vi "Highlight.vi"() -> ()   [LabVIEW 2017]
uses:
  <vilib>/Utility/traverseref.llb/TRef TravTarget.ctl
  user.lib/_NEVSTOP/Communicable State Machine(CSM)/_Polymophic/Add State(s) to Queue By BOOL(Element).vi
  user.lib/_NEVSTOP/Communicable State Machine(CSM)/Communicable State Machine.lvlib
  <vilib>/Utility/traverseref.llb/VI Scripting - Traverse.lvlib
panel:
  in  "Highlight All Scripts":bool
  in  "Highlight Scripts":bool
  out "String":string
  in  "Listbox":i32(listbox)
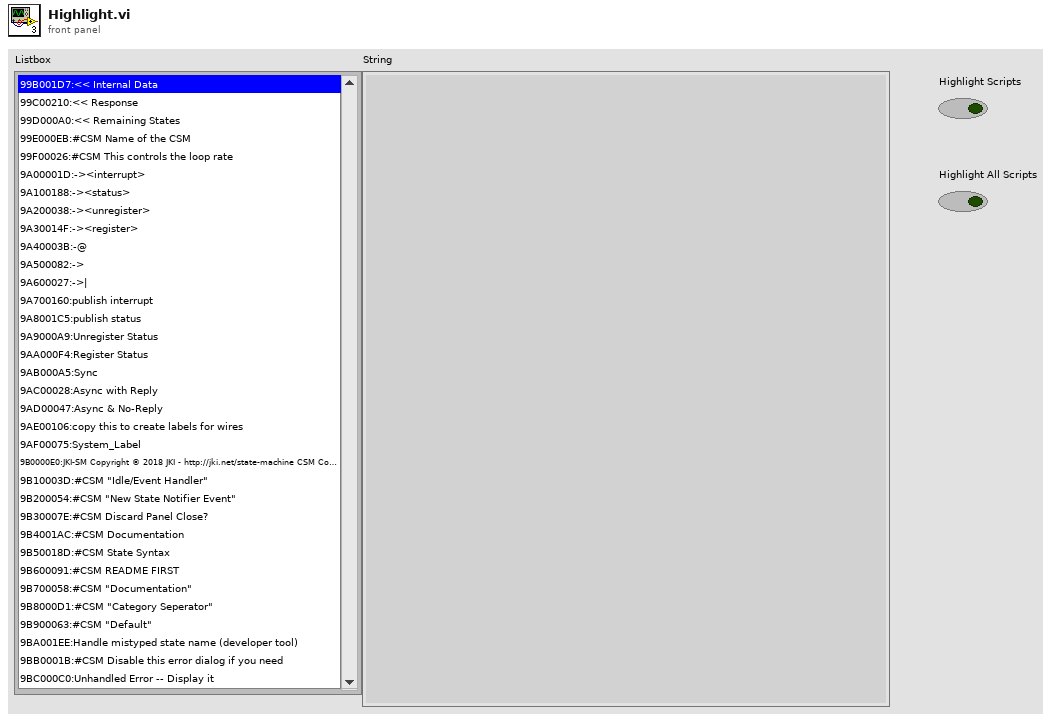
[diagram p1: front panel]
types:
  T1 = enum32{"Invalid", "Standard", "Closed", "Hidden", "Minimized", "Maximized"}
  T2 = enum32{"invalid app kind", "Development System", "Run Time System", "Student Edition", "Embedded LabVIEW", "Evaluation", "Custom"}
  T3 = typedef "TRef TravTarget.ctl" = enum16{"FP", "BD", "Other"}
  T4 = cluster{"Core":cluster{"Current VI Reference":refnum<vi>, "Close Panel on Exit?":bool}, "VI":path, "VIRef":refnum<vi>}
  T5 = cluster{"Current VI Reference":refnum<vi>, "Close Panel on Exit?":bool}
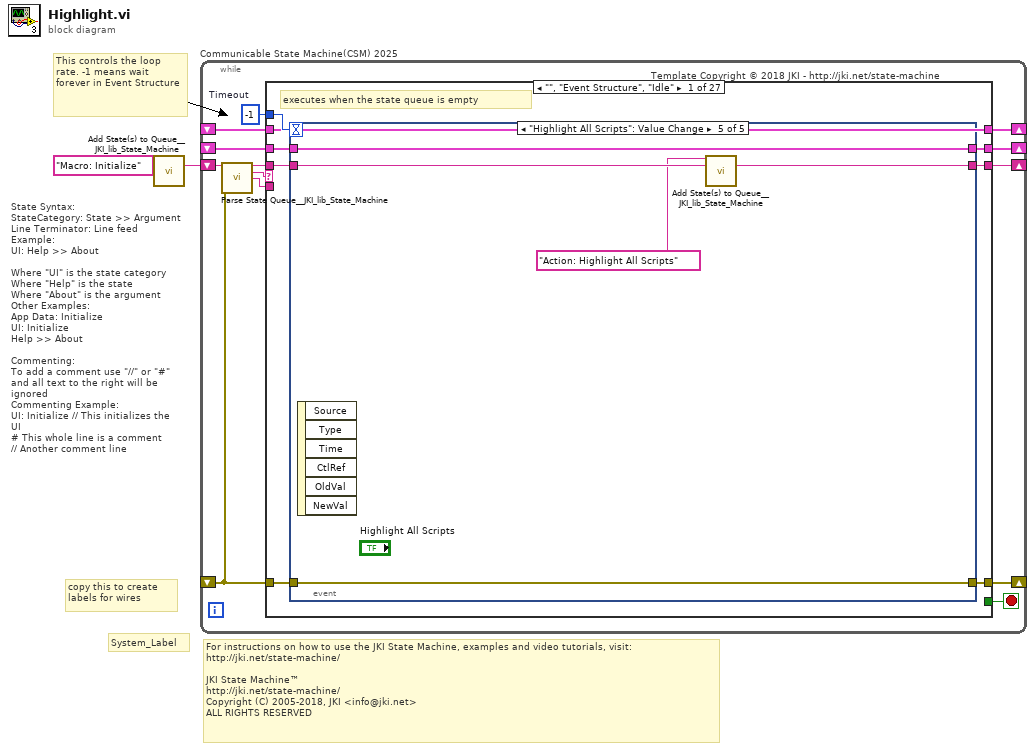
[diagram p0: block diagram]
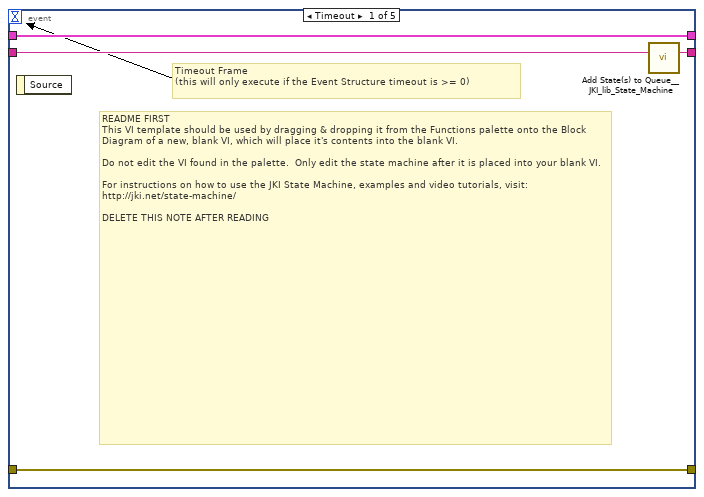
[diagram p2: hidden frame]
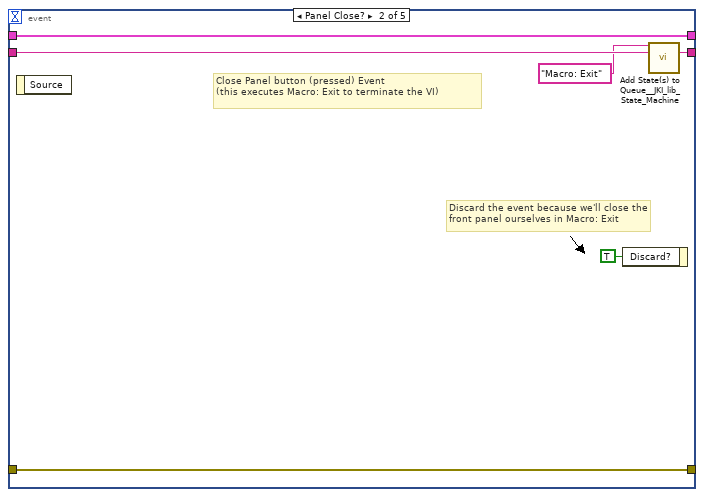
[diagram p3: hidden frame]
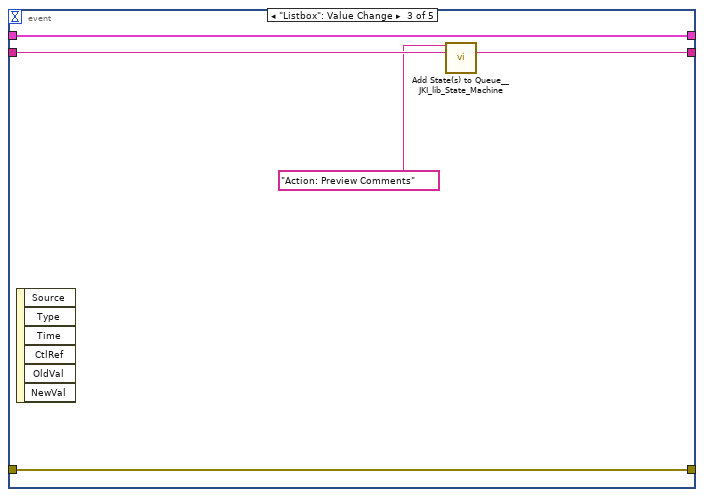
[diagram p4: hidden frame]
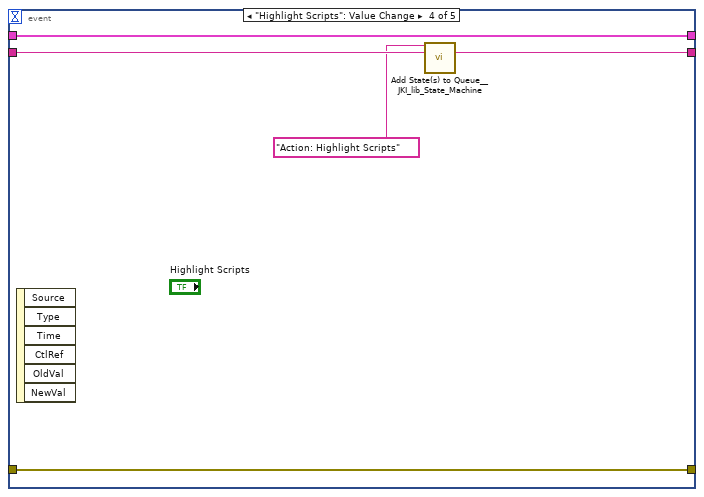
[diagram p5: hidden frame]
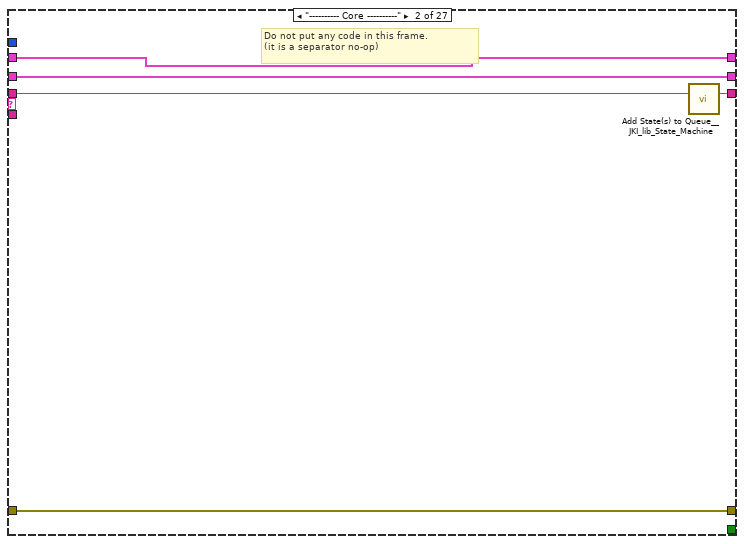
[diagram p6: hidden frame]
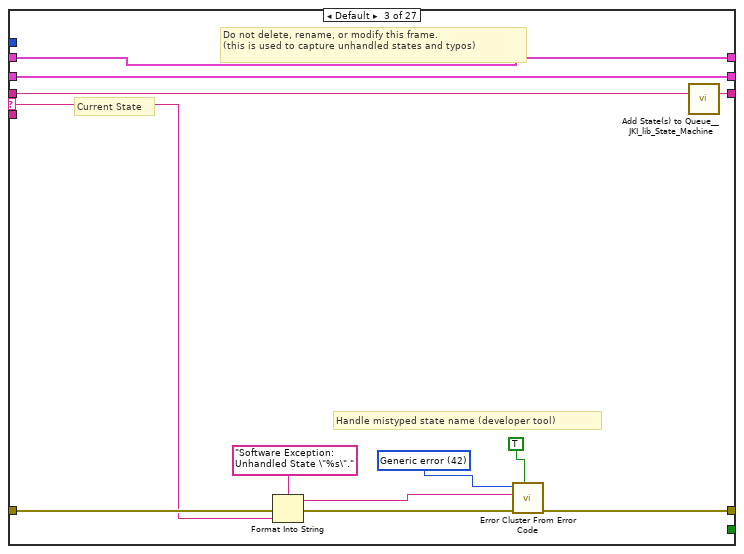
[diagram p7: hidden frame]
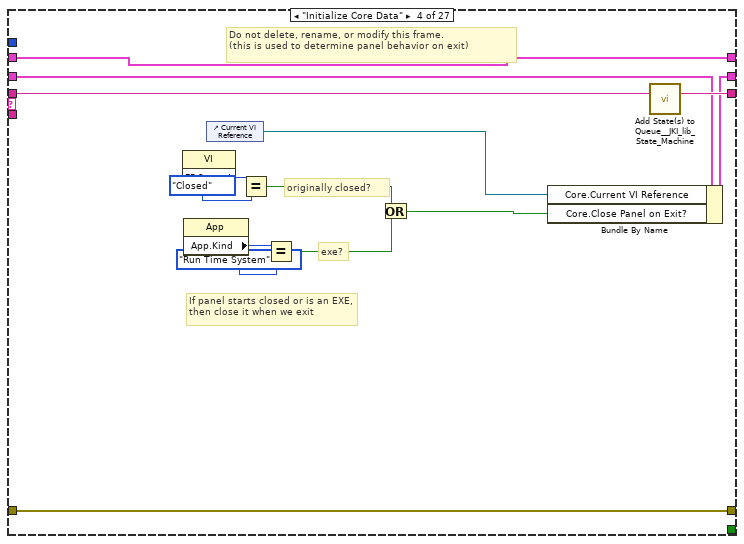
[diagram p8: hidden frame]
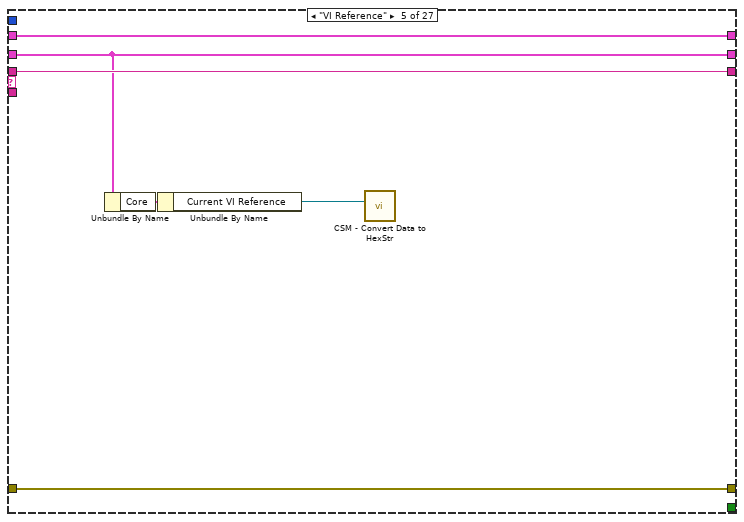
[diagram p9: hidden frame]
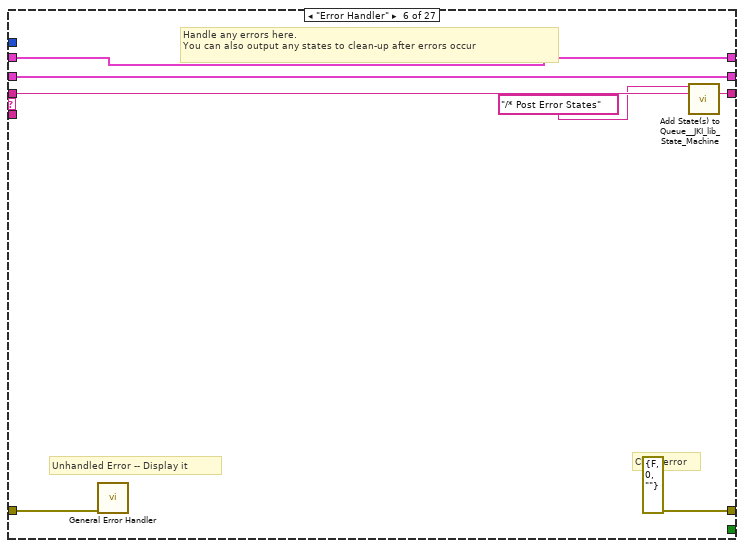
[diagram p10: hidden frame]
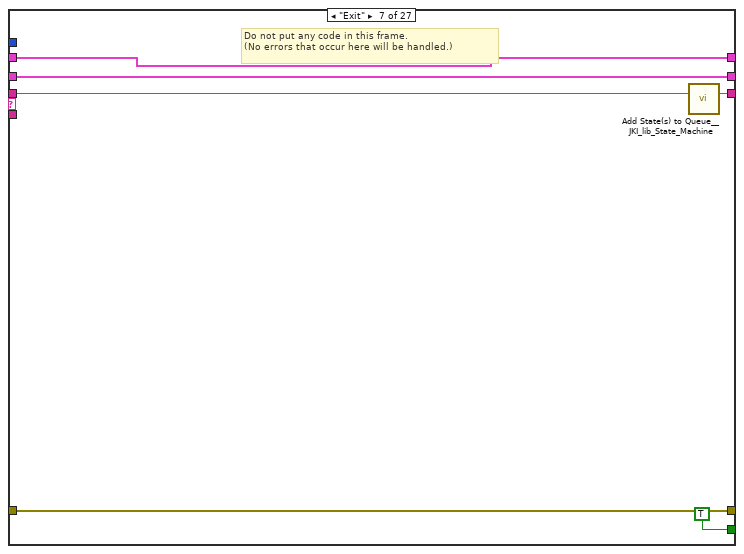
[diagram p11: hidden frame]
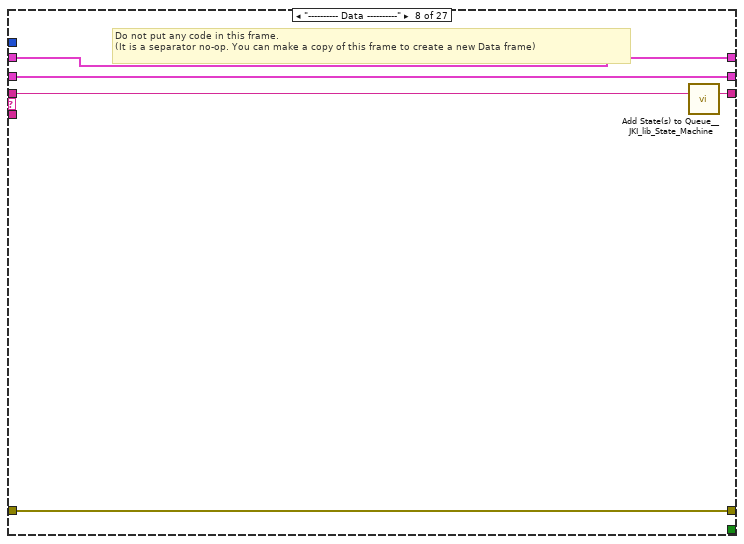
[diagram p12: hidden frame]
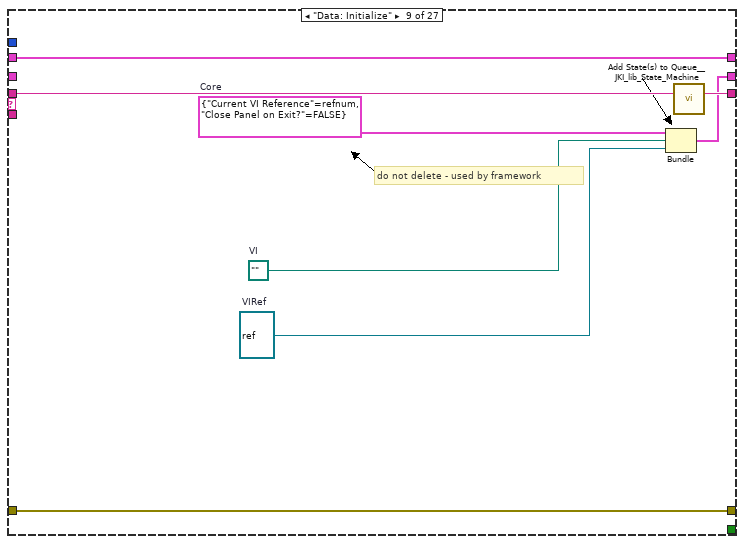
[diagram p13: hidden frame]
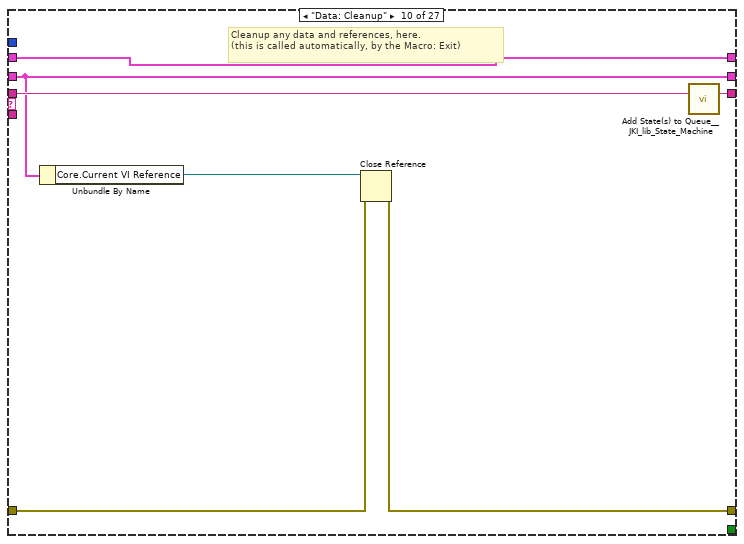
[diagram p14: hidden frame]
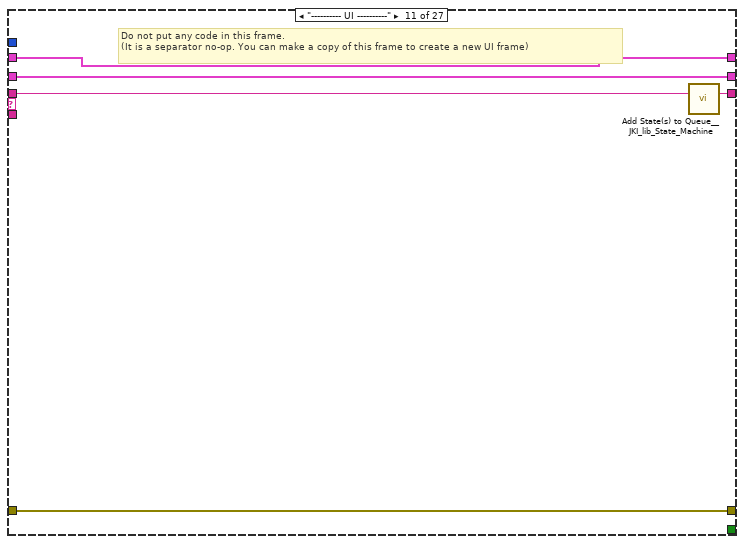
[diagram p15: hidden frame]
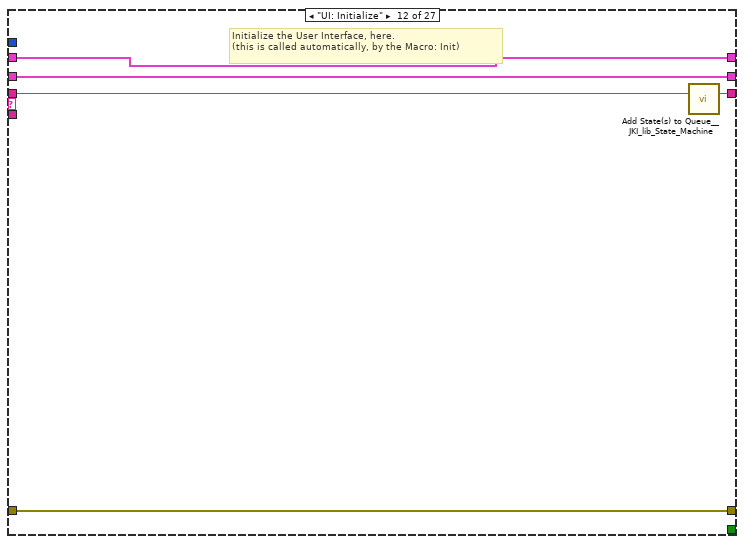
[diagram p16: hidden frame]
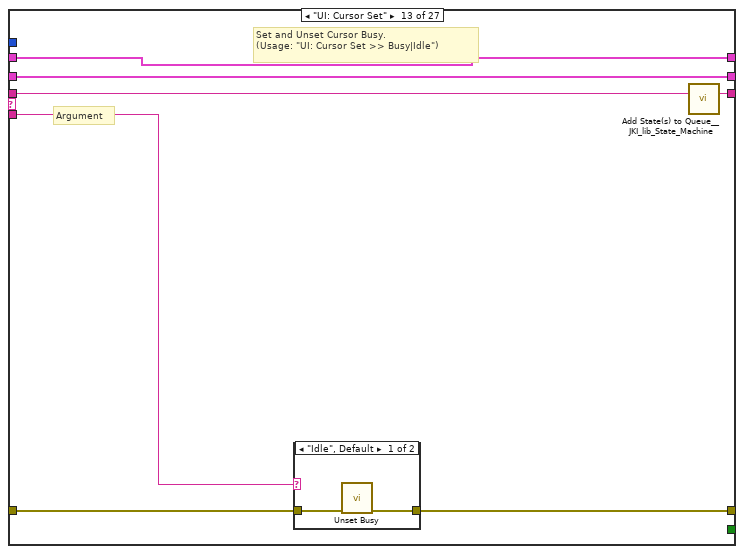
[diagram p17: hidden frame]
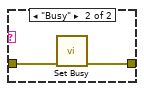
[diagram p18: hidden frame]
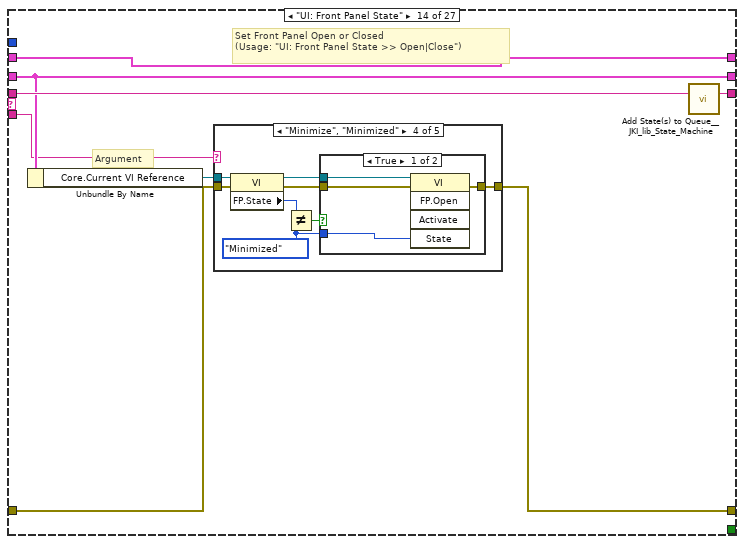
[diagram p19: hidden frame]
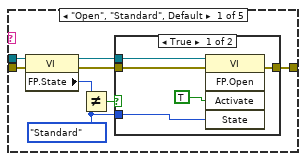
[diagram p20: hidden frame]
diagram:
  # "For instructions on how to use the JKI State Machine, examples and video tutorials, visit:\nhttp://jki.net/state-machine/\n\nJKI State Machine™\nhttp://jki.net/state-machine/\nCopyright (C) 2005-2018, JKI <info@jki.net>\nALL RIGHTS RESERVED"
  # "State Syntax:\nStateCategory: State >> Argument\nLine Terminator: Line feed\nExample:\nUI: Help >> About\n\nWhere \"UI\" is the state category\nWhere \"Help\" is the state\nWhere \"About\" is the argument\nOther Examples:\nApp Data: Initialize\nUI: Initialize\nHelp >> About\n\nCommenting:\nTo add a comment use \"//\" or \"#\" and all text to the right will be ignored\nCommenting Example:\nUI: Initialize // This initializes the UI\n# This whole line is a comment\n// Another comment line"
  # "copy this to create labels for wires"
  # "This controls the loop rate. -1 means wait forever in Event Structure"
  # "System_Label"
  n1 = call <vilib>:"Add State(s) to Queue__JKI_lib_State_Machine.vi"("State(s) in (\"\")"="Macro: Initialize") -> ("States Out"=w1:string)  [unwired: 14 in]
  n2 = while "Communicable State Machine(CSM) 2025" {
    shift-right: [w8] -> _
    shift-left: _ -> [w7]
    shift-right: [w11] -> _
    shift-left: _ -> [w5]
    shift-right: [w10] -> _
    shift-left: w1 -> [w12]
    shift-right: [w4] -> _
    shift-left: _ -> [w3]
    stop <- w9 stop-if-true
    w6 = -1  # Timeout
    # "Template Copyright © 2018 JKI - http://jki.net/state-machine"
    n3 = call <vilib>:"Parse State Queue__JKI_lib_State_Machine.vi"("State Queue"=w12, "Error In (no error)"=w5) -> ("Remaining States"=w14:string, "Current State"=w15:string, "Arguments"=w13:string)  [unwired: 11 in]
    n4 = case shown="\"\", \"Event Structure\", \"Idle\"" w15 {
      selector: w15 -> [_ _ w55 _ _ _ _ _ _ _ _ _ _ _ _ _ _ _ _ _ _ _ _ _ _ _ _]
      tunnel: w14 -> [w23 w53 w59 w79 w84 w92 w98 w103 w111 w118 w123 w128 w135 w147 w217 w223 w226 w240 w245 w257 w265 w276 w297 w311 w327 w343 w347]
      tunnel: w13 -> [_ _ _ _ _ _ _ _ _ _ _ _ w130 w141 _ _ _ _ _ _ _ _ _ _ _ _ _]
      tunnel: w7 -> [w21 w50 w57 w72 w83 w89 w96 w100 _ w113 w120 w126 w133 w143 w214 w220 w228 w237 w242 w254 w263 w275 w296 w310 w326 w342 w346]
      tunnel: [w20 w51 w61 w76 w85 errorcluster {"status"=FALSE, "code"=0, "source"=""} ("error out") w95 w101 w108 w114 w121 w125 w131 w144 w215 w221 w229 w238 w243 w255 w266 w277 w298 w312 w328 w333 w345] -> w11
      tunnel: w5 -> [w19 w51 w60 w76 w85 w88 w95 w101 w108 w115 w121 w125 w132 w145 w215 w221 w229 w238 w243 w255 w266 w277 w298 w312 w328 w333 w345]
      tunnel: [w22 w52 w58 w78 w84 w91 w97 w102 w110 w117 w122 w127 w134 w146 w216 w222 w227 w239 w244 w256 w265 w276 w297 w311 w327 w343 w347] -> w10
      tunnel: [_ _ _ _ _ _ TRUE _ _ _ _ _ _ _ _ _ _ _ _ _ _ _ _ _ _ _ _] -> w9
      tunnel: [w18 w50 w57 w77 w83 w89 w96 w100 w109 w113 w120 w126 w133 w143 w214 w220 w228 w237 w242 w248 w261 w275 w296 w310 w326 w342 w346] -> w8
      tunnel: w6 -> [w17 _ _ _ _ _ _ _ _ _ _ _ _ _ _ _ _ _ _ _ _ _ _ _ _ _ _]
      tunnel: [w16 w49 w54 w66 w82 w86 w93 w99 w104 w112 w119 w124 w129 w140 w213 w218 w224 w230 w241 w246 cluster{refnum<vi>, "Text.Text":string}[] [] w267 w287 w308 w323 w339 w344] -> w4
      tunnel: w3 -> [w16 w49 w54 w66 w82 w86 w93 w99 w104 w112 w119 w124 w129 w140 w213 w218 w224 w230 w241 w246 _ w268 w288 w308 w323 w339 w344]
      frame "", "Event Structure", "Idle" {
        # "executes when the state queue is empty"
        n5 = event shown="[4] \"Highlight All Scripts\": Value Change" {
          selector: _ -> [_ _ _ _ _]
          dyn-events: _ -> [_ _ _ _ _]
          timeout: w17 -> [_ _ _ _ _]
          tunnel: w23 -> [w27 w33 w35 w40 w45]
          tunnel: [w26 w32 w36 w41 w46] -> w22
          tunnel: w21 -> [w24 w30 w37 w42 w47]
          tunnel: [w25 w31 w38 w43 w48] -> w20
          tunnel: w19 -> [w25 w31 w38 w43 w48]
          tunnel: [w24 w30 w37 w42 w47] -> w18
          event Timeout {
            # "README FIRST\nThis VI template should be used by dragging & dropping it from the Functions palette onto the Block Diagram of a new, blank VI, which will place it's contents into the blank VI.\n\nDo not edit the VI found in the palette.  Only edit the state machine after it is placed into your blank VI.\n\nFor instructions on how to use the JKI State Machine, examples and video tutorials, visit:\nhttp://jki.net/state-machine/\n\nDELETE THIS NOTE AFTER READING"
            # "Timeout Frame\n(this will only execute if the Event Structure timeout is >= 0)"
            n6 = event-data() -> ()  [unwired: 1 in, 1 out]
            n7 = call <vilib>:"Add State(s) to Queue__JKI_lib_State_Machine.vi"("State(s) in (\"\")"=w27) -> ("States Out"=w26:string)  [unwired: 14 in]
          }
          event Panel Close? {
            # "Discard the event because we'll close the front panel ourselves in Macro: Exit"
            # "Close Panel button (pressed) Event\n(this executes Macro: Exit to terminate the VI)"
            n8 = event-data() -> ()  [unwired: 1 in, 1 out]
            n9 = event-data("Discard?"=TRUE) -> ()  [unwired: 1 in, 1 out]
            n10 = call <vilib>:"Add State(s) to Queue__JKI_lib_State_Machine.vi"("State(s) in Front (\"\")"="Macro: Exit", "State(s) in (\"\")"=w33) -> ("States Out"=w32:string)  [unwired: 13 in]
          }
          event "Listbox": Value Change {
            n11 = event-data() -> ()  [unwired: 1 in, 6 out]
            n12 = call <vilib>:"Add State(s) to Queue__JKI_lib_State_Machine.vi"("State(s) in Front (\"\")"="Action: Preview Comments" ("State(s) in Front (\"\")"), "State(s) in (\"\")"=w35) -> ("States Out"=w36:string)  [unwired: 13 in]
          }
          event "Highlight Scripts": Value Change {
            n13 = event-data() -> ()  [unwired: 1 in, 6 out]
            n14 = call <vilib>:"Add State(s) to Queue__JKI_lib_State_Machine.vi"("State(s) in Front (\"\")"="Action: Highlight Scripts" ("State(s) in Front (\"\")"), "State(s) in (\"\")"=w40) -> ("States Out"=w41:string)  [unwired: 13 in]
          }
          event "Highlight All Scripts": Value Change {
            n15 = event-data() -> ()  [unwired: 1 in, 6 out]
            n16 = call <vilib>:"Add State(s) to Queue__JKI_lib_State_Machine.vi"("State(s) in Front (\"\")"="Action: Highlight All Scripts" ("State(s) in Front (\"\")"), "State(s) in (\"\")"=w45) -> ("States Out"=w46:string)  [unwired: 13 in]
          }
        }
      }
      frame "---------- Core ----------" {
        # "Do not put any code in this frame.\n(it is a separator no-op)"
        n17 = call <vilib>:"Add State(s) to Queue__JKI_lib_State_Machine.vi"("State(s) in (\"\")"=w53) -> ("States Out"=w52:string)  [unwired: 14 in]
      }
      frame Default {
        w64 = 42 items=["No error", "Argument error", "Memory is full", "Out of zone", "End of file", "File already open", "Generic file I/O error", "File not found", "File permission error", "Disk is full", "Duplicate path", "Too many files open", "System feature not enabled", "Resource file not found", "Cannot add resource", "Resource not found", "Image not found", "Image memory error", "Pen does not exist", "Config type invalid", "Config token not found", "Config parse error", "Config memory error", "Bad external code format", "Bad external code offset", "External code not present", "Null window", "Destroy window error", "Null menu", "Print aborted", "Bad print record", "Print driver error", "Windows error during printing", "Memory error during printing", "Print dialog error", "Generic print error", "Invalid device refnum", "Device not found", "Device parameter error", "Device unit error", "Cannot open device", "Device call aborted", "Generic error", "Cancelled by user", "Object ID too low", "Object ID too high", "Object not in heap", "Unknown heap", "Unknown object (invalid DefProc)", "Unknown object (DefProc not in table)", "Message out of range", "Invalid (null) method", "Unknown message", "Manager call not supported", "Bad address", "Network operation in progress", "Network operation timed out", "Connection is busy", "Network attribute not supported", "Network error", "Address in use", "System out of memory", "Connection aborted", "Connection refused", "Not connected", "Already connected", "Connection closed", "Initialization error (interapplication manager)", "Bad occurrence", "Wait on unbound occurrence handler", "Occurrence queue overflow", "Datalog type conflict", "Unused", "Unrecognized type (interapplication manager)", "Memory corrupt", "Failed to make temporary DLL", "Old CIN version", "Drag socket not found", "Failed to load drop-object", "Failed to register OLE object", "Failed to release OLE object", "Format specifier type mismatch", "Unknown format specifier", "Too few format specifiers", "Too many format specifiers", "Scan failed", "Newer CIN version", "Error converting to variant", "Runtime menu error", "Password tampered", "Variant attribute not found", "Incompatible variant data type", "Event data is not available", "Event Store is not present", "Occurrence is not found", "Event Queue is not created", "Event info is not available", "Refnum passed is NULL", "Error retrieving Class GUID", "Error retrieving CoClass GUID", "Error retrieving TypeLib GUID.", "Bad built application magic bytes.", "Specific driver is different from the specific driver associated with the Logical Name.", "There is no session opened to the class driver.", "Max Error", "MAX - Error with config objects", "MAX - Error loading configuration", "MAX - Group not supported"]
        # "Current State"
        # "Do not delete, rename, or modify this frame.\n(this is used to capture unhandled states and typos)"
        # "Handle mistyped state name (developer tool)"
        n18 = Format Into String(format string="Software Exception: Unhandled State \"%s\"." ("message"), error in=w60, w55) -> (resulting string=w63:string, error out=w62:errorcluster)  [unwired: 1 in]
        n19 = call <vilib>:"Error Cluster From Error Code.vi"("show call chain? (False)"=TRUE, "error in (no error)"=w62, "error message (\"\")"=w63, "error code (0)"=w64) -> ("error out"=w61:errorcluster)  [unwired: 5 in]
        n20 = call <vilib>:"Add State(s) to Queue__JKI_lib_State_Machine.vi"("State(s) in (\"\")"=w59) -> ("States Out"=w58:string)  [unwired: 14 in]
      }
      frame "Initialize Core Data" {
        # "Do not delete, rename, or modify this frame.\n(this is used to determine panel behavior on exit)"
        # "originally closed?"
        # "exe?"
        # "If panel starts closed or is an EXE, then close it when we exit"
        n21 = property class="VI"() -> ("FP.State"=w69:T1)  [unwired: 2 in, 2 out]
        n22 = property class="App"() -> ("App.Kind"=w75:T2)  [unwired: 2 in, 2 out]
        n23 = control-ref of="Current VI Reference"() -> (w70:refnum<vi>)
        n24 = Equal?(x=w69, y=T1."Closed" ("Front Panel Window:State")) -> (x = y?=w67:bool)
        n25 = Equal?(x=w75, y=T2."Run Time System" ("Application:Kind")) -> (x = y?=w73:bool)
        n26 = Or(x=w67, y=w73) -> (x .or. y?=w71:bool)
        n27 = Bundle By Name(cluster=w72, "Core.Current VI Reference"=w70, "Core.Close Panel on Exit?"=w71) -> (w77:T4)
        n28 = call <vilib>:"Add State(s) to Queue__JKI_lib_State_Machine.vi"("State(s) in (\"\")"=w79) -> ("States Out"=w78:string)  [unwired: 14 in]
      }
      frame "VI Reference" {
        n29 = Unbundle By Name(w83) -> ("Core"=w81:T5)
        n30 = Unbundle By Name(w81) -> ("Current VI Reference"=w80:refnum<vi>)
        n31 = call "CSM - Convert Data to HexStr.vi"("Variant"=w80) -> ()  [unwired: 8 in, 1 out]
      }
      frame "Error Handler" {
        # "Unhandled Error -- Display it"
        # "Handle any errors here.\nYou can also output any states to clean-up after errors occur"
        # "Clear error"
        n32 = call <vilib>:"General Error Handler.vi"("error in (no error)"=w88) -> ()  [unwired: 10 in, 5 out]
        n33 = call <vilib>:"Add State(s) to Queue__JKI_lib_State_Machine.vi"("State(s) in Front (\"\")"="/* Post Error States", "State(s) in (\"\")"=w92) -> ("States Out"=w91:string)  [unwired: 13 in]
      }
      frame "Exit" {
        # "Do not put any code in this frame.\n(No errors that occur here will be handled.)"
        n34 = call <vilib>:"Add State(s) to Queue__JKI_lib_State_Machine.vi"("State(s) in (\"\")"=w98) -> ("States Out"=w97:string)  [unwired: 14 in]
      }
      frame "---------- Data ----------" {
        # "Do not put any code in this frame.\n(It is a separator no-op. You can make a copy of this frame to create a new Data frame)"
        n35 = call <vilib>:"Add State(s) to Queue__JKI_lib_State_Machine.vi"("State(s) in (\"\")"=w103) -> ("States Out"=w102:string)  [unwired: 14 in]
      }
      frame "Data: Initialize" {
        w105 = refnum<vi> refnum  # VIRef
        w106 = T5 {"Current VI Reference"=refnum, "Close Panel on Exit?"=FALSE}  # Core
        w107 = path ""  # VI
        # "do not delete - used by framework"
        n36 = Bundle("Core"=w106, "VI"=w107, "VIRef"=w105) -> (w109:T4)  [unwired: 1 in]
        n37 = call <vilib>:"Add State(s) to Queue__JKI_lib_State_Machine.vi"("State(s) in (\"\")"=w111) -> ("States Out"=w110:string)  [unwired: 14 in]
      }
      frame "Data: Cleanup" {
        # "Cleanup any data and references, here.\n(this is called automatically, by the Macro: Exit)"
        n38 = Unbundle By Name(w113) -> ("Core.Current VI Reference"=w116:refnum<vi>)
        n39 = Close Reference(reference=w116, error in (no error)=w115) -> (error out=w114:errorcluster)
        n40 = call <vilib>:"Add State(s) to Queue__JKI_lib_State_Machine.vi"("State(s) in (\"\")"=w118) -> ("States Out"=w117:string)  [unwired: 14 in]
      }
      frame "---------- UI ----------" {
        # "Do not put any code in this frame.\n(It is a separator no-op. You can make a copy of this frame to create a new UI frame)"
        n41 = call <vilib>:"Add State(s) to Queue__JKI_lib_State_Machine.vi"("State(s) in (\"\")"=w123) -> ("States Out"=w122:string)  [unwired: 14 in]
      }
      frame "UI: Initialize" {
        # "Initialize the User Interface, here.\n(this is called automatically, by the Macro: Init)"
        n42 = call <vilib>:"Add State(s) to Queue__JKI_lib_State_Machine.vi"("State(s) in (\"\")"=w128) -> ("States Out"=w127:string)  [unwired: 14 in]
      }
      frame "UI: Cursor Set" {
        # "Argument"
        # "Set and Unset Cursor Busy.\n(Usage: \"UI: Cursor Set >> Busy|Idle\")"
        n43 = case shown="\"Idle\", Default" w130 {
          tunnel: w132 -> [w137 w139]
          tunnel: [w136 w138] -> w131
          frame "Idle", Default {
            n44 = call <vilib>:"Unset Busy.vi"("error in (no error)"=w137) -> ("error out"=w136:errorcluster)  [unwired: 10 in]
          }
          frame "Busy" {
            n45 = call <vilib>:"Set Busy.vi"("error in (no error)"=w139) -> ("error out"=w138:errorcluster)  [unwired: 9 in, 1 out]
          }
        }
        n46 = call <vilib>:"Add State(s) to Queue__JKI_lib_State_Machine.vi"("State(s) in (\"\")"=w135) -> ("States Out"=w134:string)  [unwired: 14 in]
      }
      frame "UI: Front Panel State" {
        # "Argument"
        # "Set Front Panel Open or Closed\n(Usage: \"UI: Front Panel State >> Open|Close\")"
        n47 = Unbundle By Name(w143) -> ("Core.Current VI Reference"=w142:refnum<vi>)
        n48 = case shown="\"Minimize\", \"Minimized\"" w141 {
          tunnel: w145 -> [w153 w168 w179 w192 w205]
          tunnel: [w155 w169 w181 w194 w207] -> w144
          tunnel: w142 -> [w154 w166 w180 w193 w206]
          frame "Open", "Standard", Default {
            w148 = T1."Standard" ("State")
            n49 = property class="VI"(reference=w154, error in=w153) -> (reference out=w151:refnum<vi>, error out=w152:errorcluster, "FP.State"=w150:T1)
            n50 = Not Equal?(x=w150, y=w148) -> (x != y?=w149:bool)
            n51 = case shown="True" w149 {
              tunnel: [w159 w161] -> w155
              tunnel: w152 -> [w158 w161]
              tunnel: w151 -> [w157 _]
              tunnel: w148 -> [w156 _]
              frame True {
                n52 = invoke class="VI" method="FP.Open"(reference=w157, error in=w158, "Activate"=TRUE, "State"=w156) -> (error out=w159:errorcluster)  [unwired: 1 in, 4 out]
              }
              frame False {
              }
            }
          }
          frame "Close", "Closed" {
            n53 = property class="VI"(reference=w166, error in=w168) -> (reference out=w165:refnum<vi>, error out=w167:errorcluster, "FP.State"=w163:T1)
            n54 = Not Equal?(x=w163, y=T1."Closed" ("Front Panel Window:State")) -> (x != y?=w162:bool)
            n55 = case shown="True" w162 {
              tunnel: [w170 w173] -> w169
              tunnel: w167 -> [w170 w172]
              tunnel: w165 -> [_ w171]
              frame False {
              }
              frame True {
                n56 = invoke class="VI" method="FP.Close"(reference=w171, error in=w172) -> (error out=w173:errorcluster)  [unwired: 1 in, 2 out]
              }
            }
          }
          frame "Hidden", "Hide" {
            w174 = T1."Hidden" ("State")
            n57 = property class="VI"(reference=w180, error in=w179) -> (reference out=w177:refnum<vi>, error out=w178:errorcluster, "FP.State"=w176:T1)
            n58 = Not Equal?(x=w176, y=w174) -> (x != y?=w175:bool)
            n59 = case shown="True" w175 {
              tunnel: [w185 w186] -> w181
              tunnel: w178 -> [w184 w186]
              tunnel: w177 -> [w183 _]
              tunnel: w174 -> [w182 _]
              frame True {
                n60 = invoke class="VI" method="FP.Open"(reference=w183, error in=w184, "State"=w182) -> (error out=w185:errorcluster)  [unwired: 2 in, 4 out]
              }
              frame False {
              }
            }
          }
          frame "Minimize", "Minimized" {
            w187 = T1."Minimized" ("State")
            n61 = property class="VI"(reference=w193, error in=w192) -> (reference out=w190:refnum<vi>, error out=w191:errorcluster, "FP.State"=w189:T1)
            n62 = Not Equal?(x=w189, y=w187) -> (x != y?=w188:bool)
            n63 = case shown="True" w188 {
              tunnel: [w198 w199] -> w194
              tunnel: w191 -> [w197 w199]
              tunnel: w190 -> [w196 _]
              tunnel: w187 -> [w195 _]
              frame True {
                n64 = invoke class="VI" method="FP.Open"(reference=w196, error in=w197, "State"=w195) -> (error out=w198:errorcluster)  [unwired: 2 in, 4 out]
              }
              frame False {
              }
            }
          }
          frame "Maximize", "Maximized" {
            w200 = T1."Maximized" ("State")
            n65 = property class="VI"(reference=w206, error in=w205) -> (reference out=w203:refnum<vi>, error out=w204:errorcluster, "FP.State"=w202:T1)
            n66 = Not Equal?(x=w202, y=w200) -> (x != y?=w201:bool)
            n67 = case shown="True" w201 {
              tunnel: [w211 w212] -> w207
              tunnel: w204 -> [w210 w212]
              tunnel: w203 -> [w209 _]
              tunnel: w200 -> [w208 _]
              frame True {
                n68 = invoke class="VI" method="FP.Open"(reference=w209, error in=w210, "State"=w208) -> (error out=w211:errorcluster)  [unwired: 2 in, 4 out]
              }
              frame False {
              }
            }
          }
        }
        n69 = call <vilib>:"Add State(s) to Queue__JKI_lib_State_Machine.vi"("State(s) in (\"\")"=w147) -> ("States Out"=w146:string)  [unwired: 14 in]
      }
      frame "---------- Macro ----------" {
        # "Do not put any code in this frame.\n(It is a separator no-op. You can make a copy of this frame to create a new Macro frame)"
        n70 = call <vilib>:"Add State(s) to Queue__JKI_lib_State_Machine.vi"("State(s) in (\"\")"=w217) -> ("States Out"=w216:string)  [unwired: 14 in]
      }
      frame "Macro: Initialize" {
        w219 = "Data: Initialize\nInitialize Core Data\nUI: Initialize\nUI: Front Panel State >> Open\n//\nAction: Load VI"  # Data: Initialize Initialize Core Data UI: Initialize UI: Front Panel State >> Open // Action: Load VI
        # "Initialization Macro\n(This is called once, when the VI starts)"
        n71 = call <vilib>:"Add State(s) to Queue__JKI_lib_State_Machine.vi"("State(s) in Front (\"\")"=w219, "State(s) in (\"\")"=w223) -> ("States Out"=w222:string)  [unwired: 13 in]
      }
      frame "Macro: Script" {
        n72 = call <vilib>:"Add State(s) to Queue__JKI_lib_State_Machine.vi"("State(s) in Front (\"\")"="Action: OpenVI\nAction: Load Text Decor\nAction: Load StringConstant\nAction: Update UI" ("State(s) in Front (\"\")"), "State(s) in (\"\")"=w226) -> ("States Out"=w227:string)  [unwired: 13 in]
      }
      frame "Macro: Exit" {
        # "Exit Macro\n(This is called once, when the VI exits)"
        n73 = Unbundle By Name(w237) -> ("Core.Close Panel on Exit?"=w236:bool)
        n74 = Select(t="UI: Front Panel State >> Close", s=w236, f="") -> (s? t:f=w233:string)
        n75 = call <vilib>:"Add State(s) to Queue__JKI_lib_State_Machine.vi"("State(s) in (\"\")"=w233, "State(s) at Back (\"\")"="Data: Cleanup\nExit") -> ("States Out"=w231:string)  [unwired: 13 in]
        n76 = call <vilib>:"Add State(s) to Queue__JKI_lib_State_Machine.vi"("State(s) in Front (\"\")"=w231, "State(s) in (\"\")"=w240) -> ("States Out"=w239:string)  [unwired: 13 in]
      }
      frame "---------- Action ----------" {
        # "Template Separator\n(You can make a copy of, or modify, this frame)"
        n77 = call <vilib>:"Add State(s) to Queue__JKI_lib_State_Machine.vi"("State(s) in (\"\")"=w245) -> ("States Out"=w244:string)  [unwired: 14 in]
      }
      frame "Action: Load VI" {
        n78 = call "File Dialog"("pattern (all files)"="*.vi") -> ("selected path"=w247:path, "error out"=w252:errorcluster)  [unwired: 11 in, 2 out]
        n79 = Not(x=w252) -> (.not. x?=w251:bool)
        n80 = Bundle By Name(cluster=w254, "VI"=w247) -> (w248:T4)
        n81 = call-poly "Add State(s) to Queue By BOOL++.vi"("FALSE (\"\")"="Macro: Exit" ("pattern (all files)"), "TRUE (\"\")"="Macro: Script" ("pattern (all files)"), "Condition"=w251, "State Queue (\"\")"=w257) -> ("Remaining States"=w256:string)  [unwired: 7 in]
      }
      frame "Action: OpenVI" {
        n82 = Unbundle By Name(w263) -> ("VI"=w262:path)
        n83 = Open VI Reference(vi path=w262, options=2) -> (vi reference=w259:refnum<vi>)  [unwired: 4 in, 1 out]
        n84 = invoke class="VI" method="FP.Open"(reference=w259) -> (reference out=w260:refnum<vi>)  [unwired: 4 in, 4 out]
        n85 = Bundle By Name(cluster=w263, "VIRef"=w260) -> (w261:T4)
      }
      frame "Action: Load Text Decor" {
        n86 = Unbundle By Name(w275) -> ("VIRef"=w269:refnum<vi>)
        n87 = call <vilib>:"Traverse for GObjects.vi"("Traverse Target"=TRef_TravTarget."BD", "Class Name"="Text", "VI Refnum"=w269) -> ("error out"=w270:errorcluster, "References"=w272:refnum<vi>[])  [unwired: 5 in, 2 out]
        n88 = for {
          tunnel: w272 -> [w278] mode=indexing
          tunnel: w270 -> [w286]
          tunnel: [w283] -> w271 mode=indexing if=w281
          n89 = To More Specific Class(target class=refnum<vi> refnum ("reference out"), reference=w278, error in=w286) -> (specific class reference=w285:refnum<vi>, error out=w284:errorcluster)
          n90 = property class="Txt"(reference=w285, error in=w284) -> (error out=w282:errorcluster, "Text"=w280:string)  [unwired: 1 out]
          n91 = Not(x=w282) -> (.not. x?=w281:bool)
          n92 = Bundle(w278, "Text"=w280) -> (w283:cluster{refnum<vi>, "Text":string})  [unwired: 1 in]
        }
        n93 = Build Array (concatenate)(w268, w271) -> (w267:cluster{refnum<vi>, "Text":string}[])
      }
      frame "Action: Load StringConstant" {
        n94 = Unbundle By Name(w296) -> ("VIRef"=w290:refnum<vi>)
        n95 = call <vilib>:"Traverse for GObjects.vi"("Traverse Target"=TRef_TravTarget."BD", "Class Name"="StringConstant", "VI Refnum"=w290) -> ("error out"=w291:errorcluster, "References"=w293:refnum<vi>[])  [unwired: 5 in, 2 out]
        n96 = for {
          tunnel: w293 -> [w299] mode=indexing
          tunnel: w291 -> [w307]
          tunnel: [w304] -> w292 mode=indexing if=w302
          tunnel: refnum<vi> refnum ("reference out") -> [w300]
          n97 = To More Specific Class(target class=w300, reference=w299, error in=w307) -> (specific class reference=w306:refnum<vi>, error out=w305:errorcluster)
          n98 = property class="StrCnst"(reference=w306, error in=w305) -> (error out=w303:errorcluster, "Text.Text"=w301:string)  [unwired: 1 out]
          n99 = Not(x=w303) -> (.not. x?=w302:bool)
          n100 = Bundle(w299, "Text.Text"=w301) -> (w304:cluster{refnum<vi>, "Text.Text":string})  [unwired: 1 in]
        }
        n101 = Build Array (concatenate)(w288, w292) -> (w287:cluster{refnum<vi>, "Text.Text":string}[])
      }
      frame "Action: Update UI" {
        n102 = for {
          tunnel: w308 -> [w321] mode=indexing
          tunnel: [w313] -> w309 mode=indexing
          w315 = u32 0  # U32
          n103 = Unbundle(w321) -> (w317:refnum<vi>, "Text.Text"=w320:string)
          n104 = call "CSM - Break Down Multiple States String.vi"("States"=w320) -> ("Multiple States"=w319:string[])  [unwired: 10 in]
          n105 = Type Cast(type=w315, x=w317) -> (*(type *) &x=w314:u32)
          n106 = Index Array(array=w319) -> (element=w318:string)  [unwired: 1 in]
          n107 = Format Into String(format string="%x:%s", w314, w318) -> (resulting string=w313:string)  [unwired: 2 in, 1 out]
        }
        n108 = property on="Listbox" class="LstBox (strict)"("Item Names"=w309) -> ()  [unwired: 2 in, 2 out]
      }
      frame "Action: Preview Comments" {
        n109 = Index Array(array=w323, index="Listbox") -> (element=w324:cluster{refnum<vi>, "Text.Text":string})
        n110 = Unbundle(w324) -> ("Text.Text"=→"String":string)  [unwired: 1 out]
      }
      frame "Action: Highlight Scripts" {
        n111 = local read "Listbox"() -> (w341:i32)
        n112 = Index Array(array=w339, index=w341) -> (element=w340:cluster{refnum<vi>, "Text.Text":string})
        n113 = Unbundle(w340) -> (w335:refnum<vi>)  [unwired: 1 out]
        n114 = To More Specific Class(target class=refnum<vi> refnum ("reference out"), reference=w335) -> (specific class reference=w337:refnum<vi>, error out=w330:errorcluster)  [unwired: 1 in]
        n115 = To More Specific Class(target class=refnum<vi> refnum ("reference out"), reference=w335) -> (specific class reference=w334:refnum<vi>, error out=w329:errorcluster)  [unwired: 1 in]
        n116 = call "_Highlight CSM Scripts(TextDecor).vi"("error in (no error)"=w330, "Reference Out 2"=w337) -> ("error out"=w331:errorcluster)  [unwired: 9 in]
        n117 = call "_Highlight CSM Scripts(StringConstant).vi"("error in (no error)"=w329, "Reference Out"=w334) -> ("error out"=w332:errorcluster)  [unwired: 9 in]
        n118 = call <vilib>:"Clear Errors.vi"("error in (no error)"=w331) -> ()  [unwired: 5 in, 2 out]
        n119 = call <vilib>:"Clear Errors.vi"("error in (no error)"=w332) -> ()  [unwired: 5 in, 2 out]
      }
      frame "Action: Highlight All Scripts" {
        n120 = for {
          tunnel: w344 -> [w348] mode=indexing
          n121 = Unbundle(w348) -> (w354:refnum<vi>)  [unwired: 1 out]
          n122 = To More Specific Class(target class=refnum<vi> refnum ("reference out"), reference=w354) -> (specific class reference=w356:refnum<vi>, error out=w350:errorcluster)  [unwired: 1 in]
          n123 = To More Specific Class(target class=refnum<vi> refnum ("reference out"), reference=w354) -> (specific class reference=w353:refnum<vi>, error out=w349:errorcluster)  [unwired: 1 in]
          n124 = call "_Highlight CSM Scripts(TextDecor).vi"("error in (no error)"=w350, "Reference Out 2"=w356) -> ("error out"=w351:errorcluster)  [unwired: 9 in]
          n125 = call "_Highlight CSM Scripts(StringConstant).vi"("error in (no error)"=w349, "Reference Out"=w353) -> ("error out"=w352:errorcluster)  [unwired: 9 in]
          n126 = call <vilib>:"Clear Errors.vi"("error in (no error)"=w351) -> ()  [unwired: 5 in, 2 out]
          n127 = call <vilib>:"Clear Errors.vi"("error in (no error)"=w352) -> ()  [unwired: 5 in, 2 out]
        }
      }
    }
  }
